vi "写入Last Reading.vi"(8 "error in (no error)":errorcluster caption="错误输入（无错误）", 10 "Last Reading":dbl, 11 "Sensor输入":refnum<class "Sensor.lvclass">) -> (0 "error out":errorcluster caption="错误输出", 3 "Sensor输出":refnum<class "Sensor.lvclass">)   [LabVIEW 2026, in "Sensor.lvclass"]
doc: "Writes one field of this class's private data. Generated by lvai_create_accessors from the class private data control."
uses:
  Sensor.lvclass
  Sensor.lvclass/Sensor.ctl
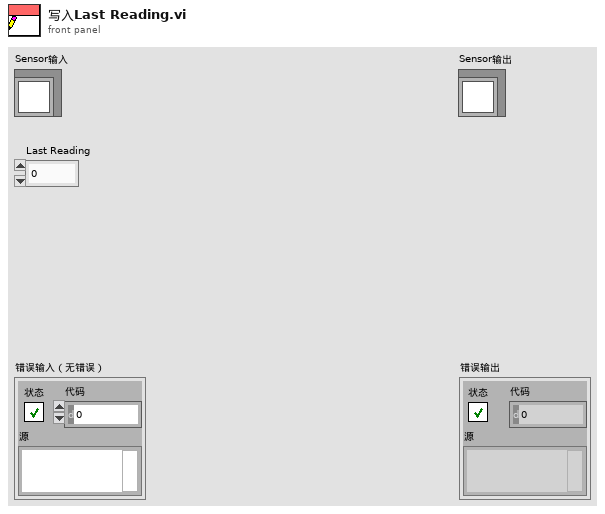
[diagram p1: front panel]
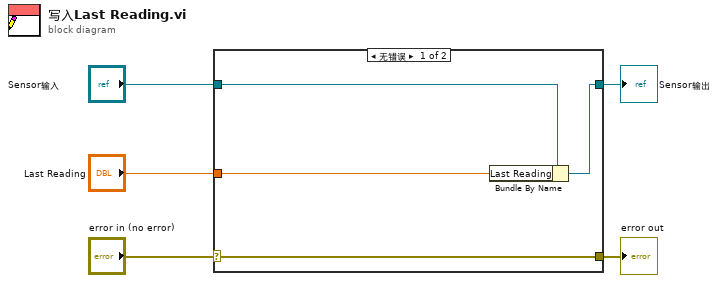
[diagram p0: block diagram]
diagram:
  n1 = case shown="无错误" "error in (no error)" {
    selector: "error in (no error)" -> [w9 w10]
    tunnel: [w9 w10] -> w4
    tunnel: [w7 w11] -> w2
    tunnel: "Sensor输入" -> [w8 w11]
    tunnel: "Last Reading" -> [w6 _]
    frame No Error {
      n2 = Bundle By Name(cluster=w8, "Last Reading"=w6) -> (w7:refnum<class "Sensor.lvclass">)
    }
    frame Error {
    }
  }
  "error out" <- w4
  "Sensor输出" <- w2
